vi "Invalid Venv Path--error.vi"() -> (0 "error out":errorcluster)   [LabVIEW 2026]
doc: "Invalid path to virtual environment. This could signalize an attempt of code injection."
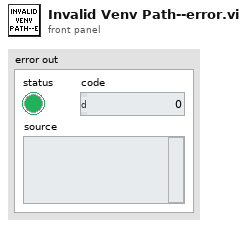
[diagram p1: front panel]
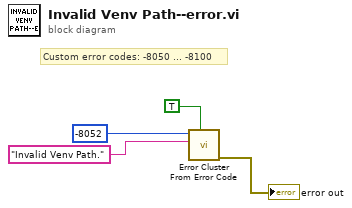
[diagram p0: block diagram]
diagram:
  # "Custom error codes: -8050 ... -8100"
  n1 = call <vilib>:"Error Cluster From Error Code.vi"("show call chain? (False)"=TRUE, "error message (\"\")"="Invalid Venv Path." ("error message (\"\")"), "error code (0)"=-8052) -> ("error out"=→"error out":errorcluster)  [unwired: 6 in]
